vi "Integ.Time To Fps.vi"(11 "integrationTimes (us)":dbl[](array[numeric])) -> (3 "fps string":string[](array[string]))   [LabVIEW 2025, in "VarexWrapper.lvlib"]
uses:
  VarexWrapper.lvlib
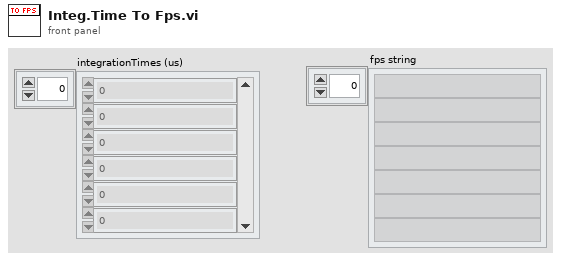
[diagram p1: front panel]
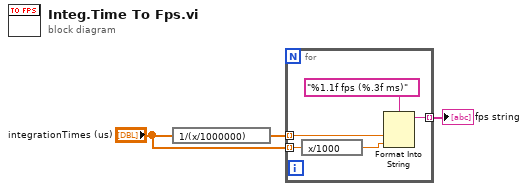
[diagram p0: block diagram]
diagram:
  n1 = expression code="1/(x/1000000)"("integrationTimes (us)") -> (w3:dbl[])
  n2 = for {
    tunnel: w3 -> [w6] mode=indexing
    tunnel: [w7] -> w1 mode=indexing
    tunnel: "integrationTimes (us)" -> [w5] mode=indexing
    n3 = expression code="x/1000"(w5) -> (w4:dbl)
    n4 = Format Into String(format string="%1.1f fps (%.3f ms)", w6, w4) -> (resulting string=w7:string)  [unwired: 2 in, 1 out]
  }
  "fps string" <- w1
